vi "ControllerUI_New_with_command_read.vi"() -> ()   [LabVIEW 2026]
uses:
  <vilib>/Utility/error.llb/Trim Whitespace One-Sided.vi
panel:
  out "Numeric":i32
  out "after substring":string
  out "String":string
  out "script Status 3":string caption="script Status"
  out "script Status 2":string caption="script Status"
  in  "Percentage":dbl(slide) step=1.0 scale=0.0..100.0 scale format="%#.6g"
  out "IP":string="192.168.149.128"
  out "Port":dbl
  in  "BTN_DESD_3":bool
  in  "BTN_Grid_1":bool
  in  "BTN_Load_4":bool
  in  "BTN_Load_2":bool
  in  "BTN_Load_3":bool
  in  "BTN_Load_1":bool
  in  "BTN_DESD_2":bool
  in  "BTN_Gen_1":bool
  in  "BTN_PV_1":bool
  in  "BTN_Gen_2":bool
  in  "BTN_PV_2":bool
  in  "BTN_DESD_4":bool
  in  "BTN_DESD_1":bool
  in  "BTN_Wind_Turbine":bool
  out "background":picture
  in  "Tab Control":T1(tab)
  in  "Mode 4":bool
  in  "Mode 3":bool
  in  "Mode 2":bool
  in  "Mode 1：5-Day Rainstorm-to-Flood":bool
  out "script Status":string
  out "remaining text":string
  in  "String Control":string
  in  "PA1":dbl caption="Percentage (0-100)" min=0.0 max=30.0 step=0.5
  in  "stop":bool
  out "Local Status":string
  in  "PA3":dbl caption="Voltage 2 (0-255)" min=0.0 max=255.0 step=1.0
  out "Last Update":string
  out "UDP Frame":string
  out "Active Power":string
  out "Current":string
  out "Voltage":string
  in  "Reset Node":bool
  in  "Read Device State":bool
  in  "Send UDP Command":bool
  in  "PA2":dbl caption="Voltage 1 (0-255)" min=0.0 max=80.0 step=1.0
  in  "Voltage Command":dbl min=0.0 max=255.0 step=1.0
  in  "Node Enable":bool
  out "Device Badge":string
  out "Selected Summary":string
  out "Device Description":string
  out "Node ID":string
  out "Device Name":string
  # "Preset Disaster Mode"
  # "Selected Node Telemetry"
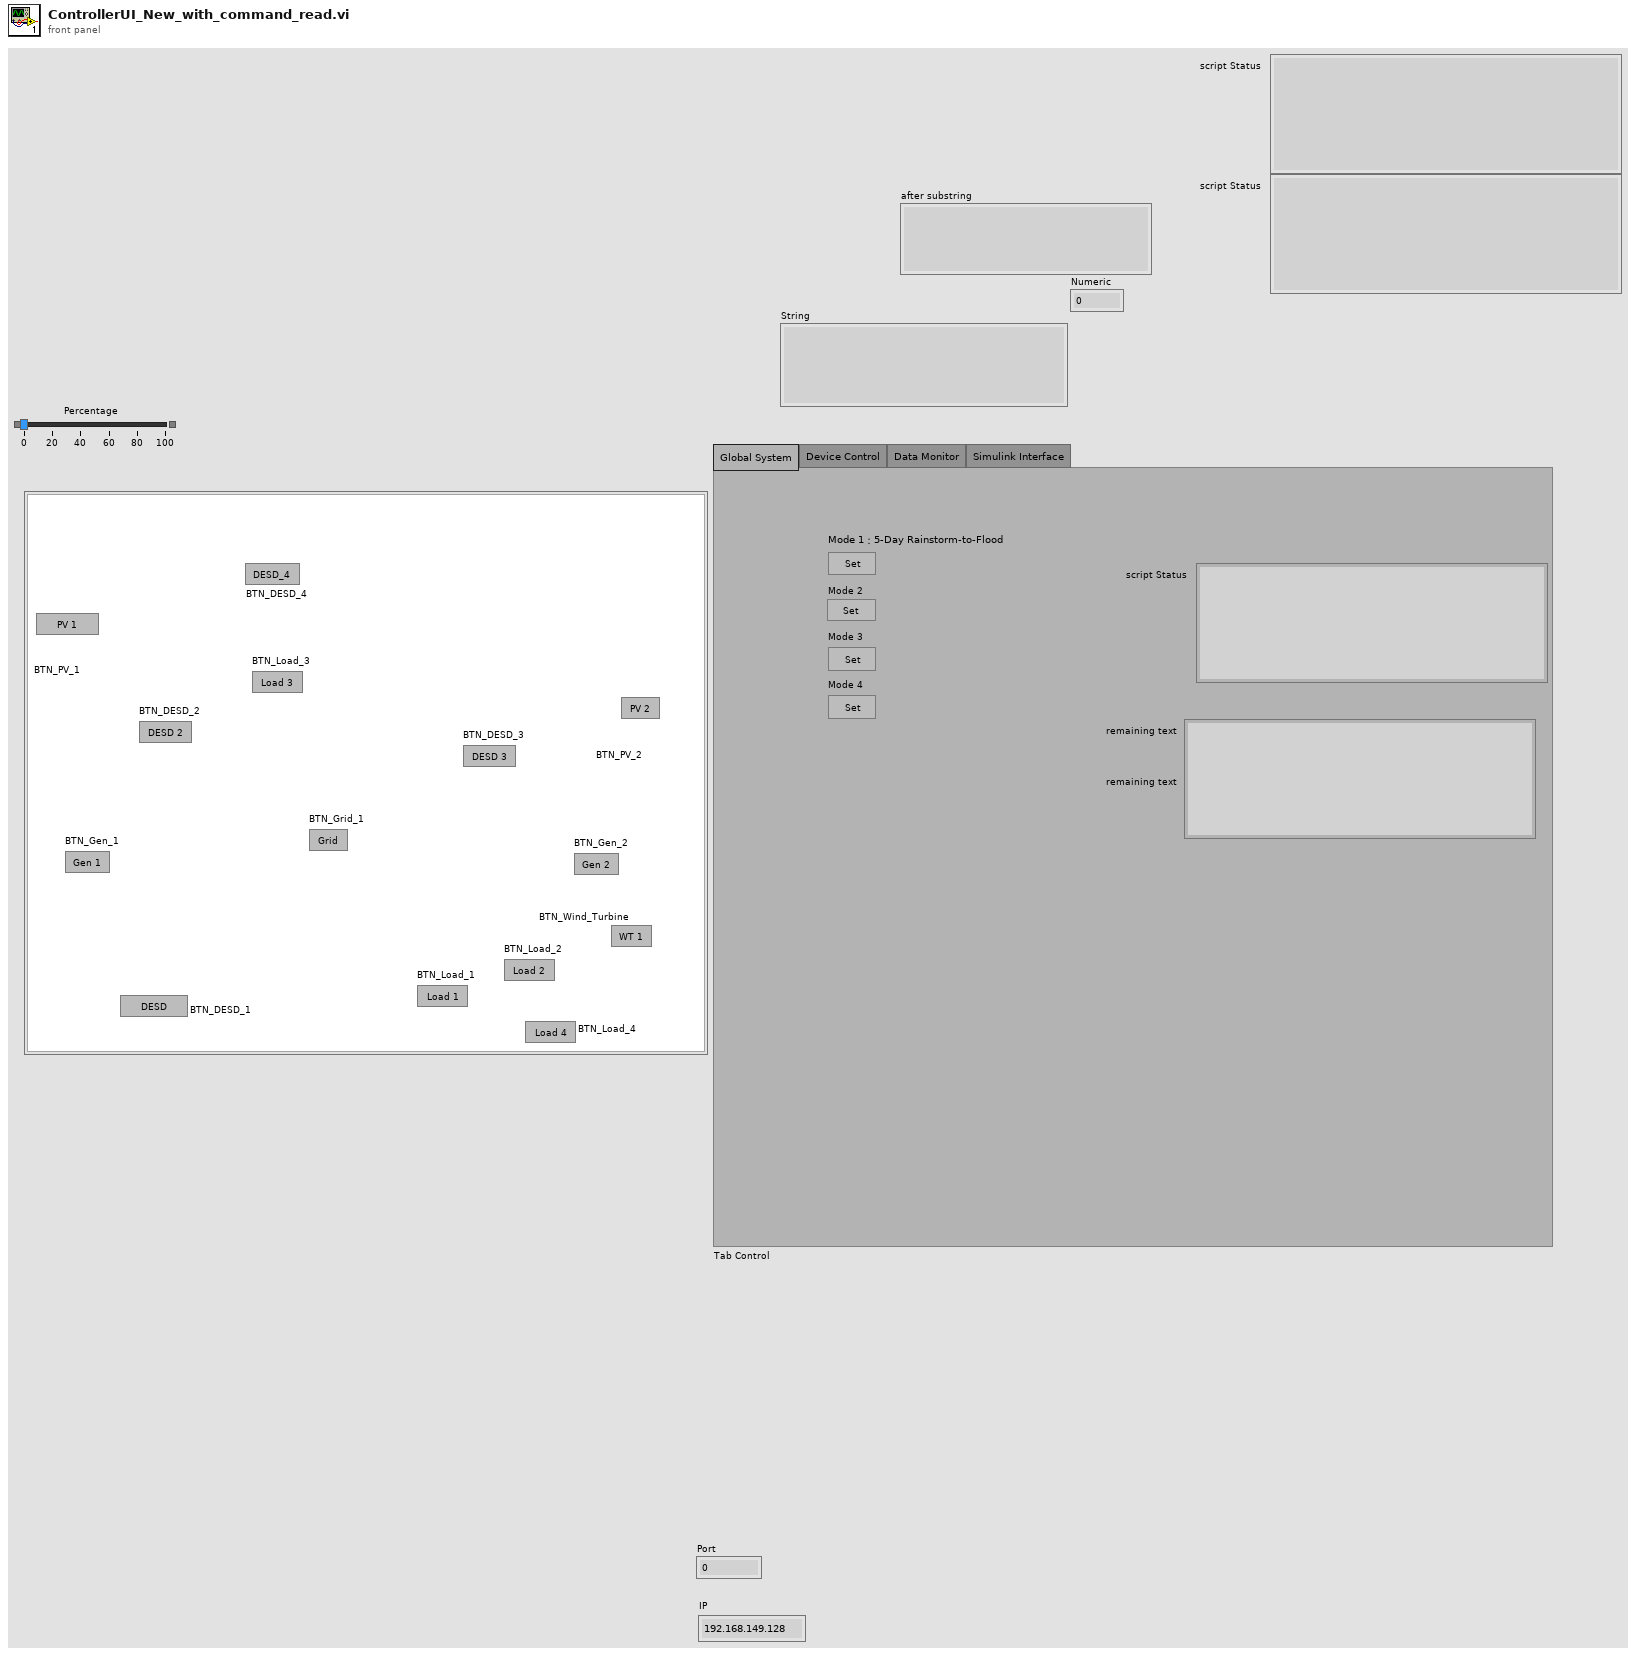
[diagram p1: front panel]
types:
  T1 = enum32{"Global System", "Device Control", "Data Monitor", "Simulink Interface"}
  T2 = typedef "imagedata.ctl" = cluster{"image type":i32, "image depth":i32, "image":u8[], "mask":u8[], "colors":u32[], "Rectangle":cluster{"left":i16, "top":i16, "right":i16, "bottom":i16}}
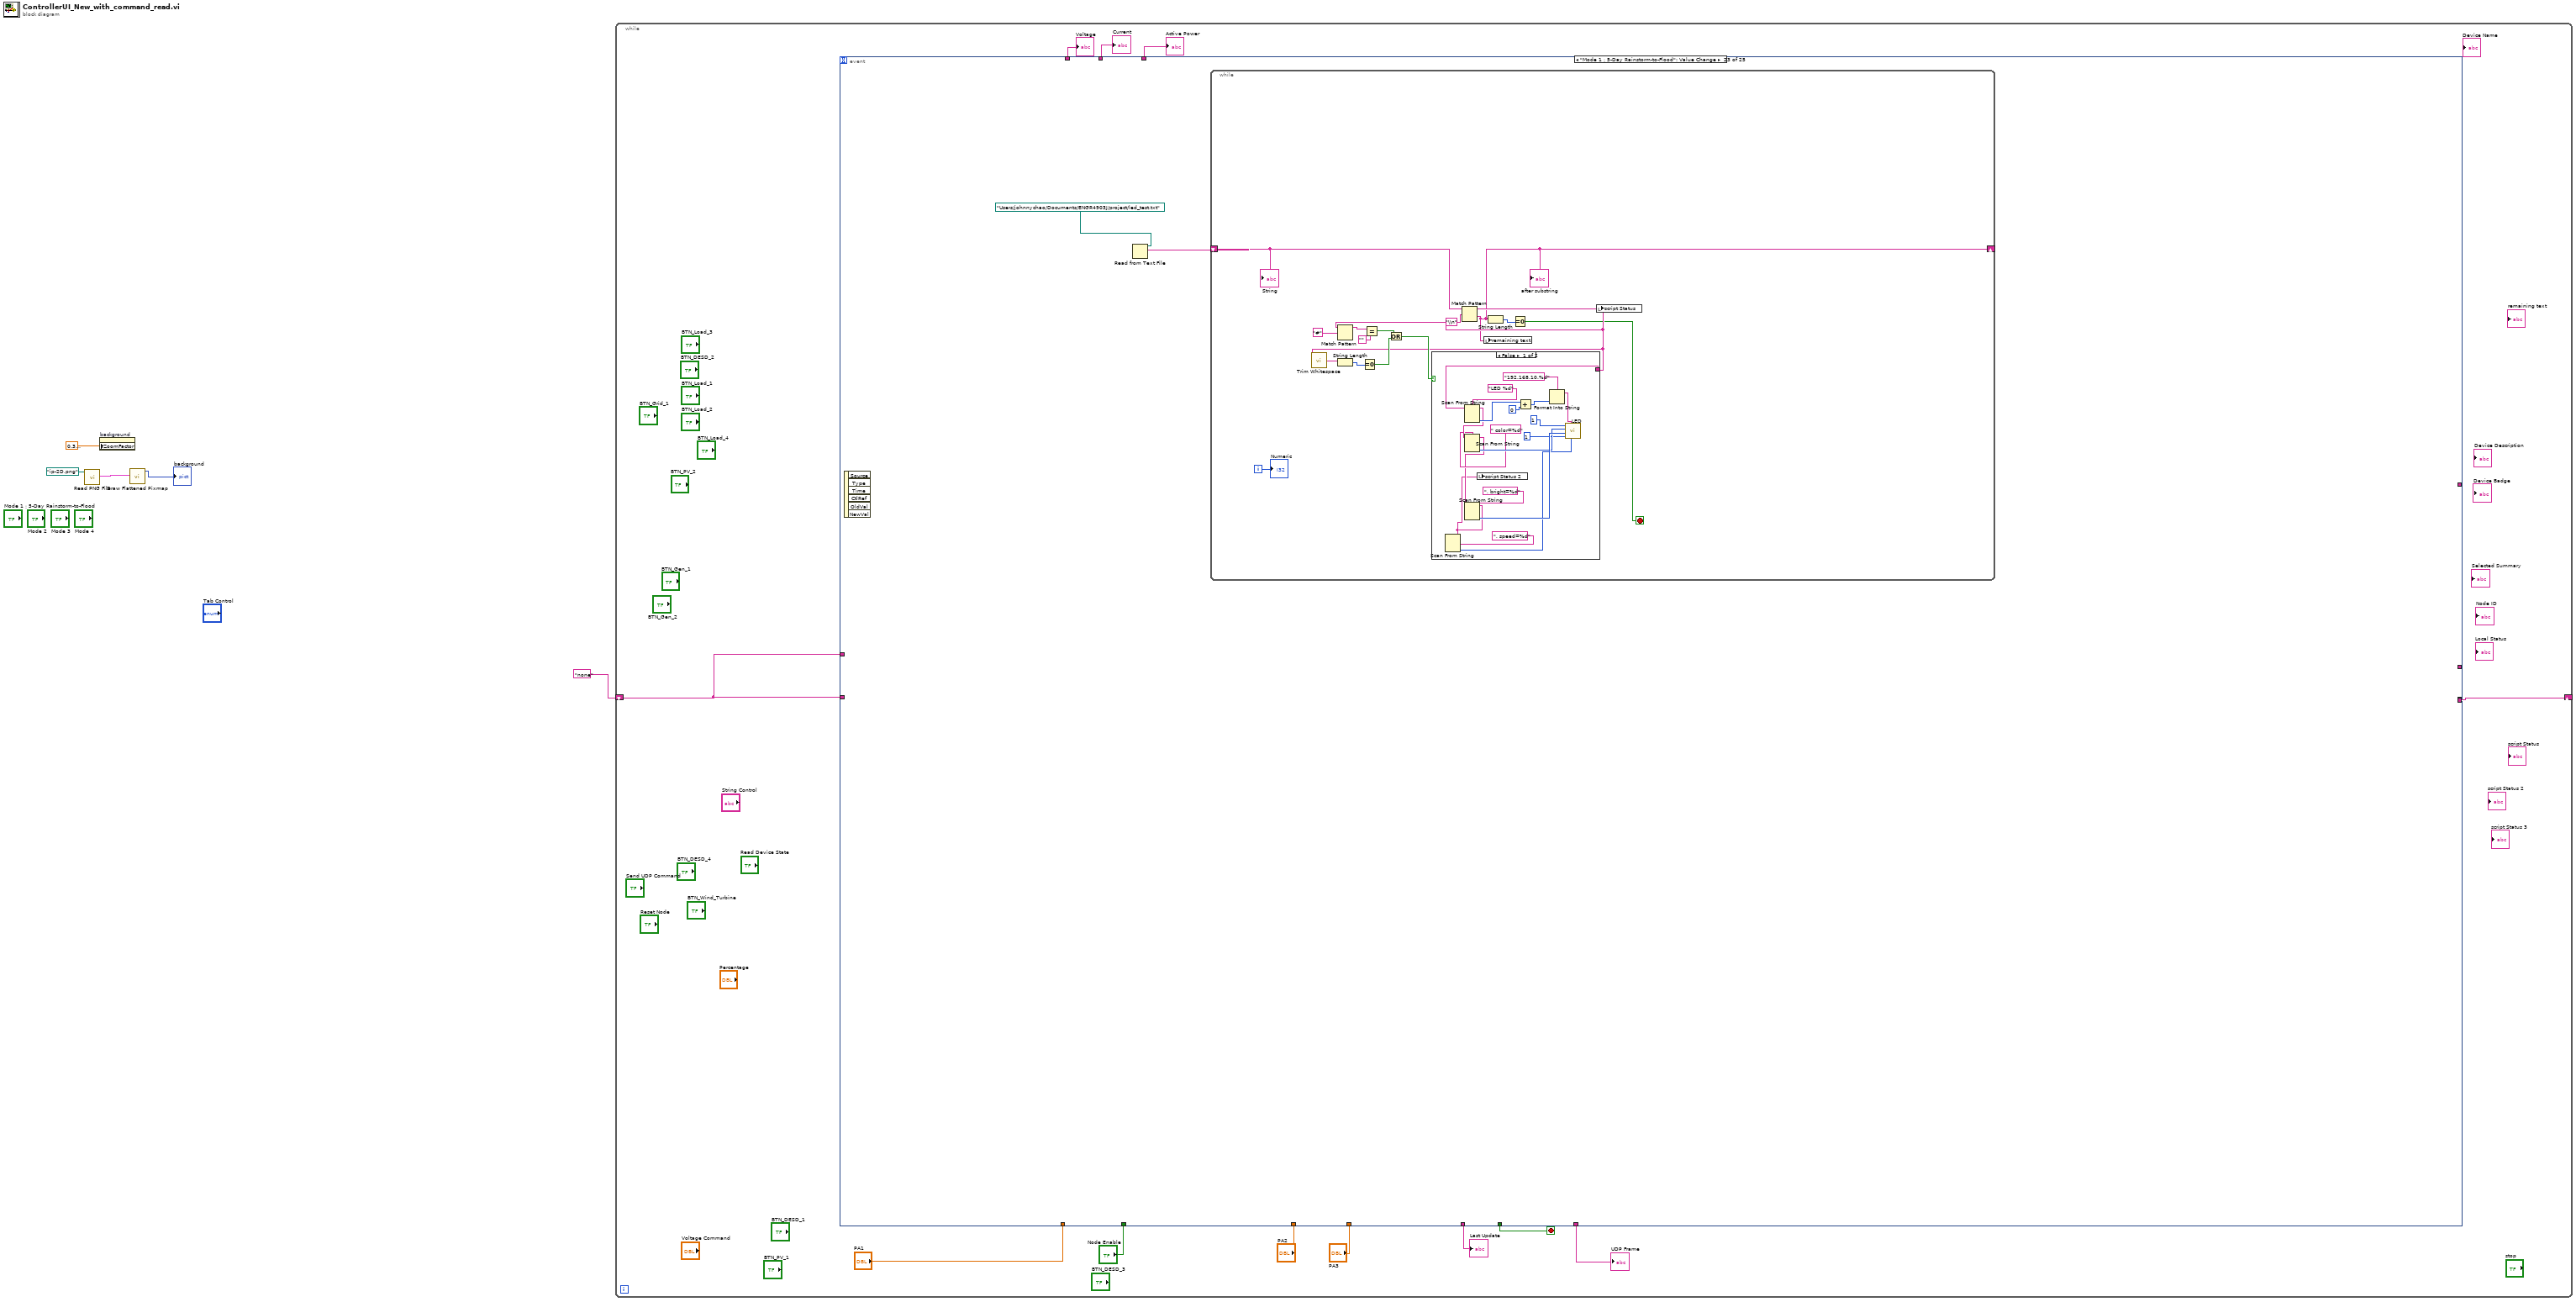
[diagram p0: block diagram]
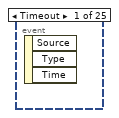
[diagram p2: hidden frame]
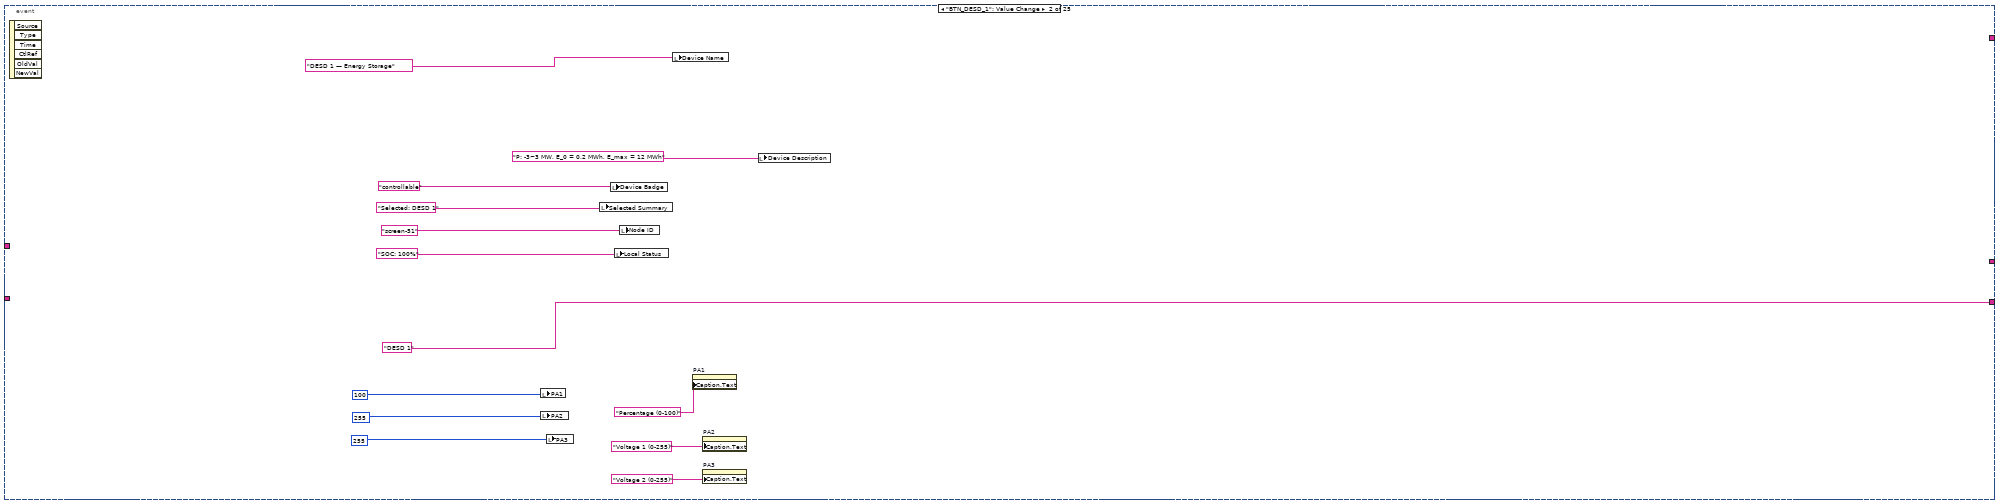
[diagram p3: hidden frame]
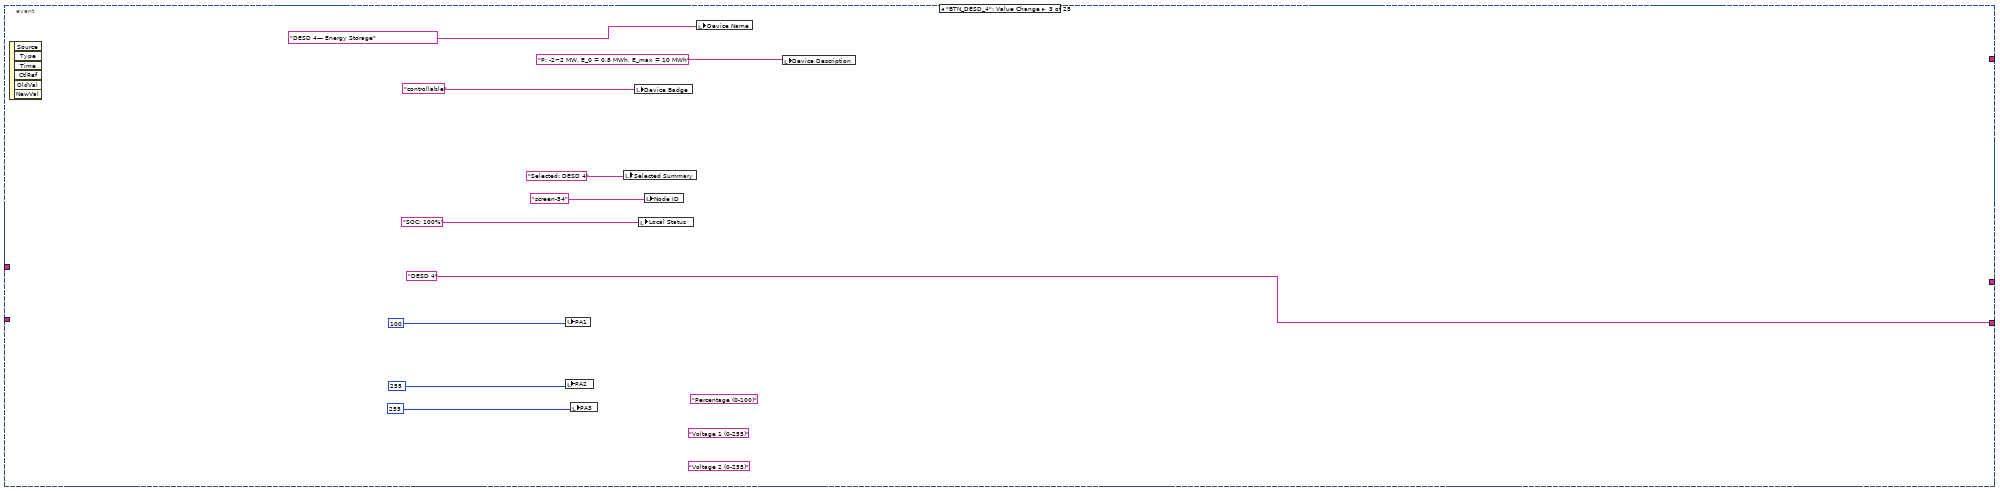
[diagram p4: hidden frame]
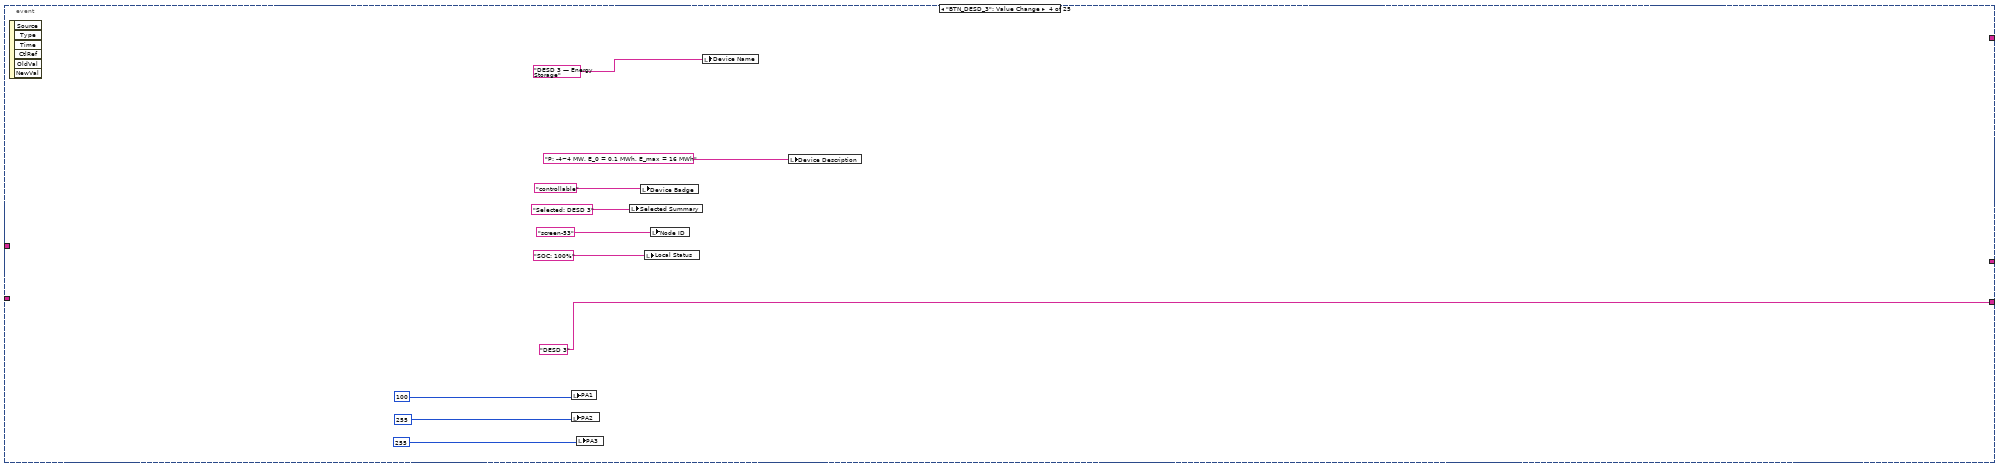
[diagram p5: hidden frame]
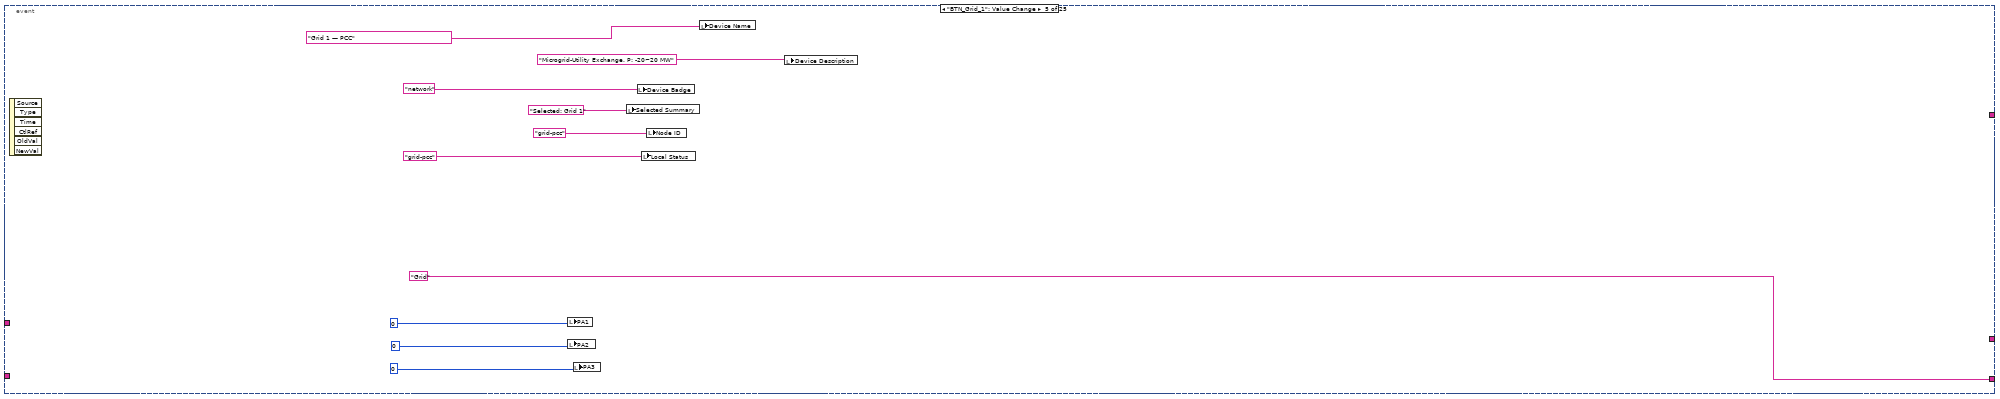
[diagram p6: hidden frame]
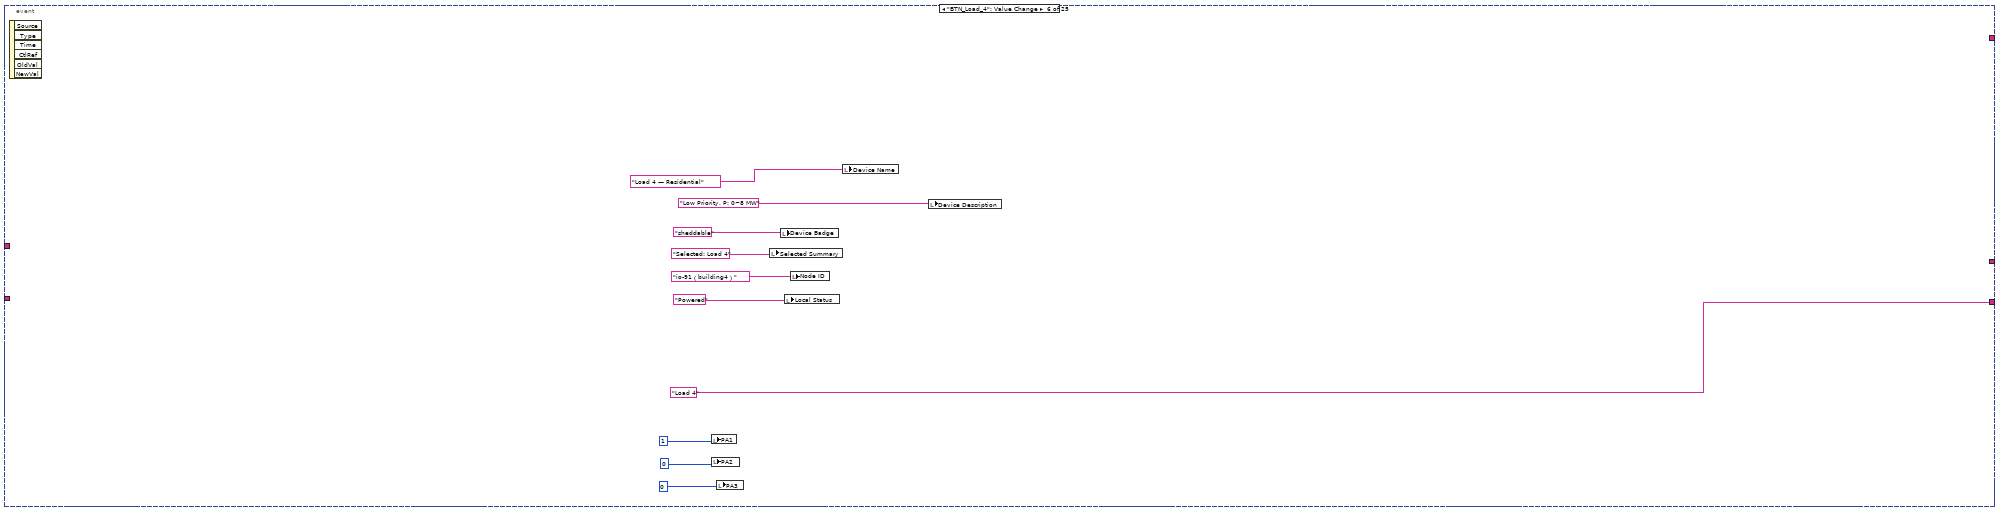
[diagram p7: hidden frame]
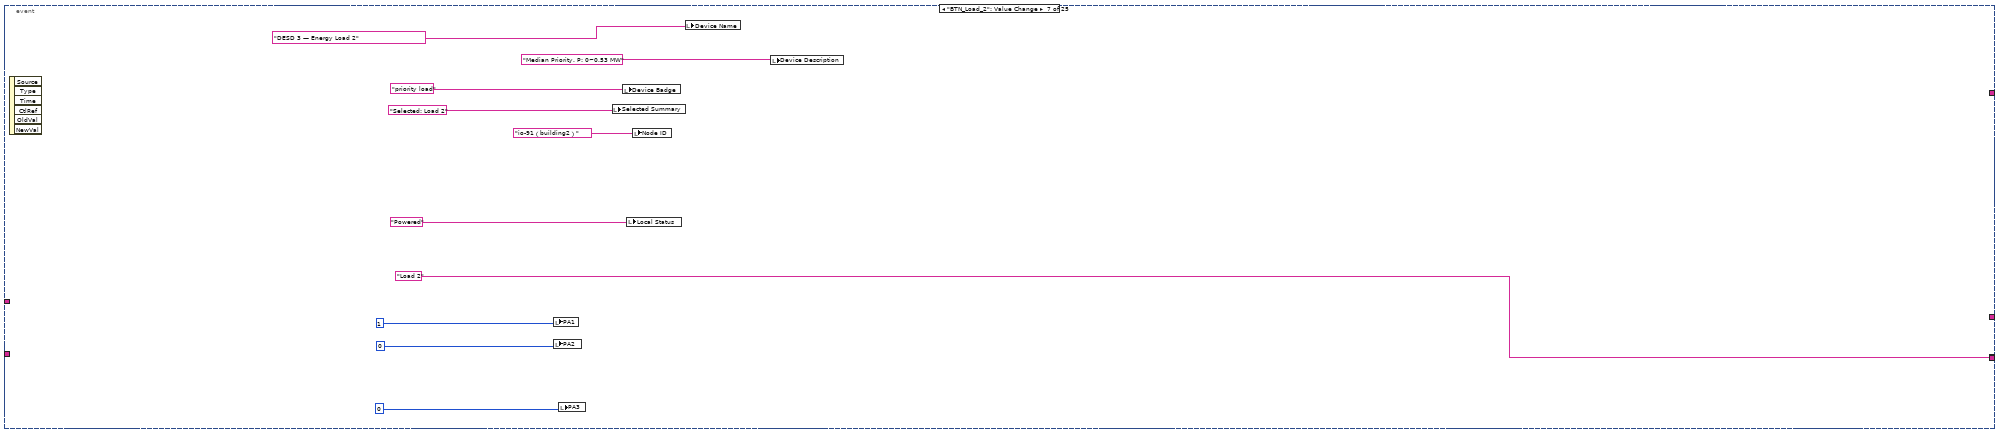
[diagram p8: hidden frame]
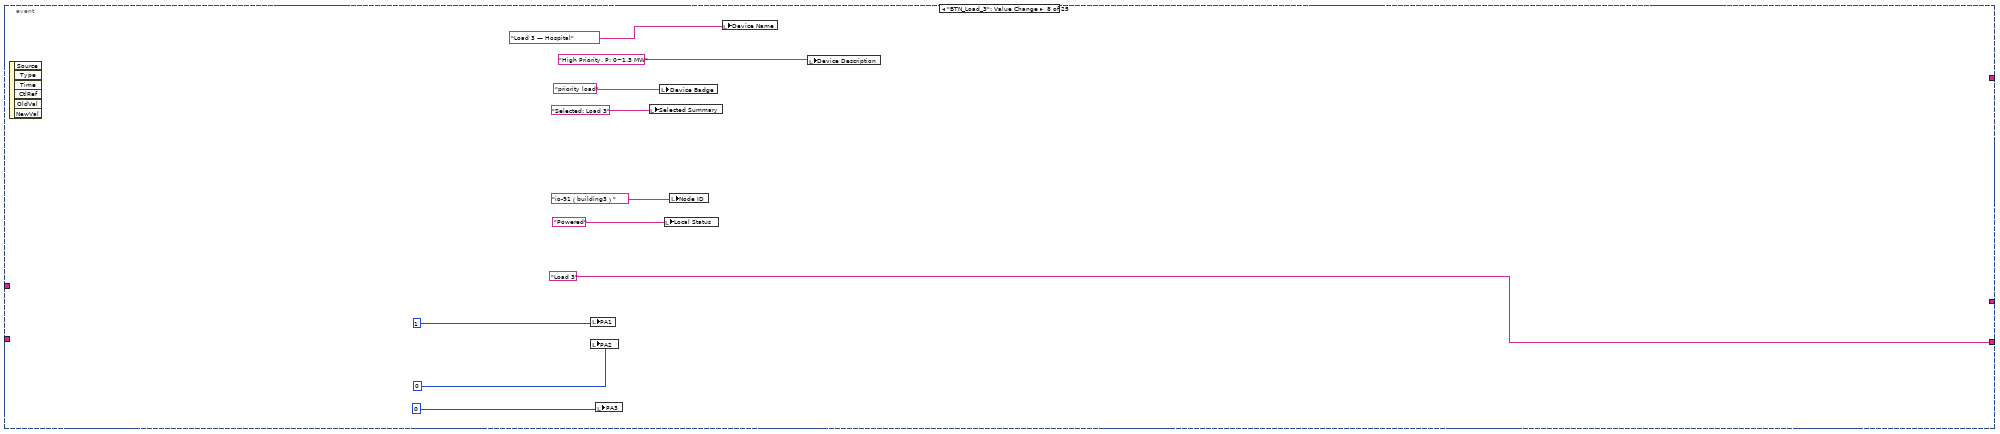
[diagram p9: hidden frame]
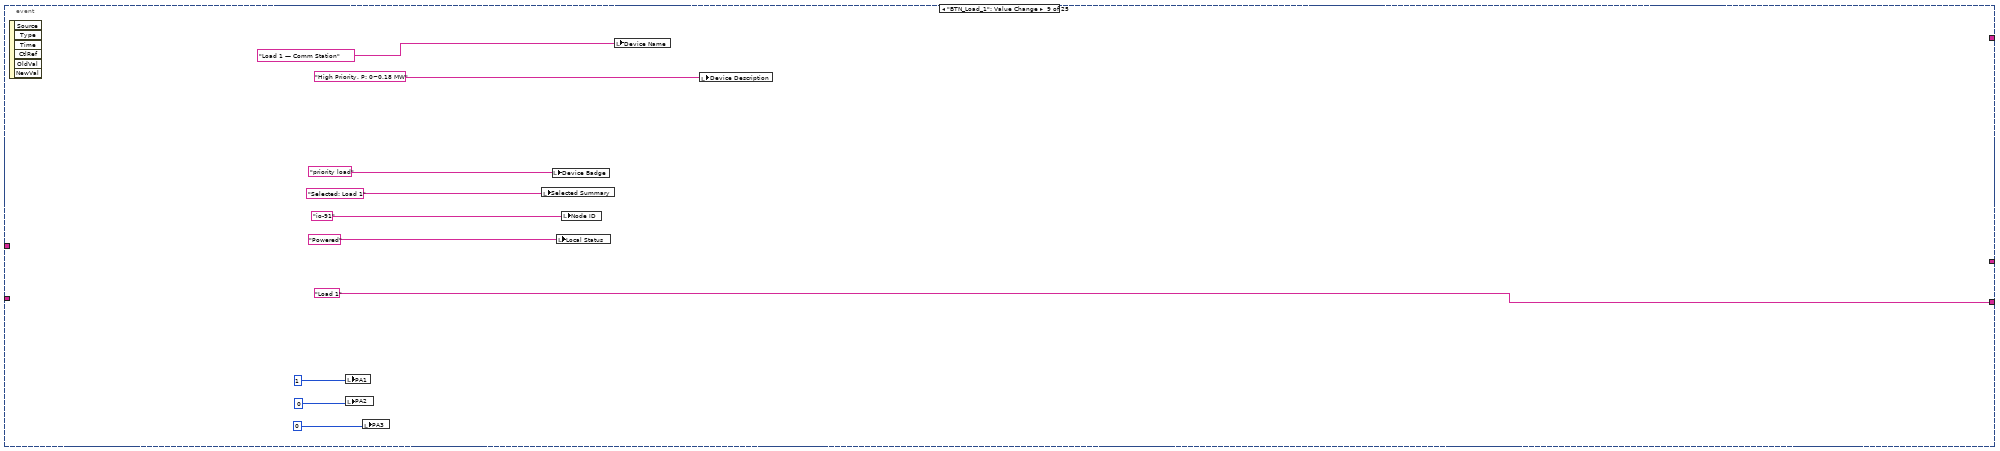
[diagram p10: hidden frame]
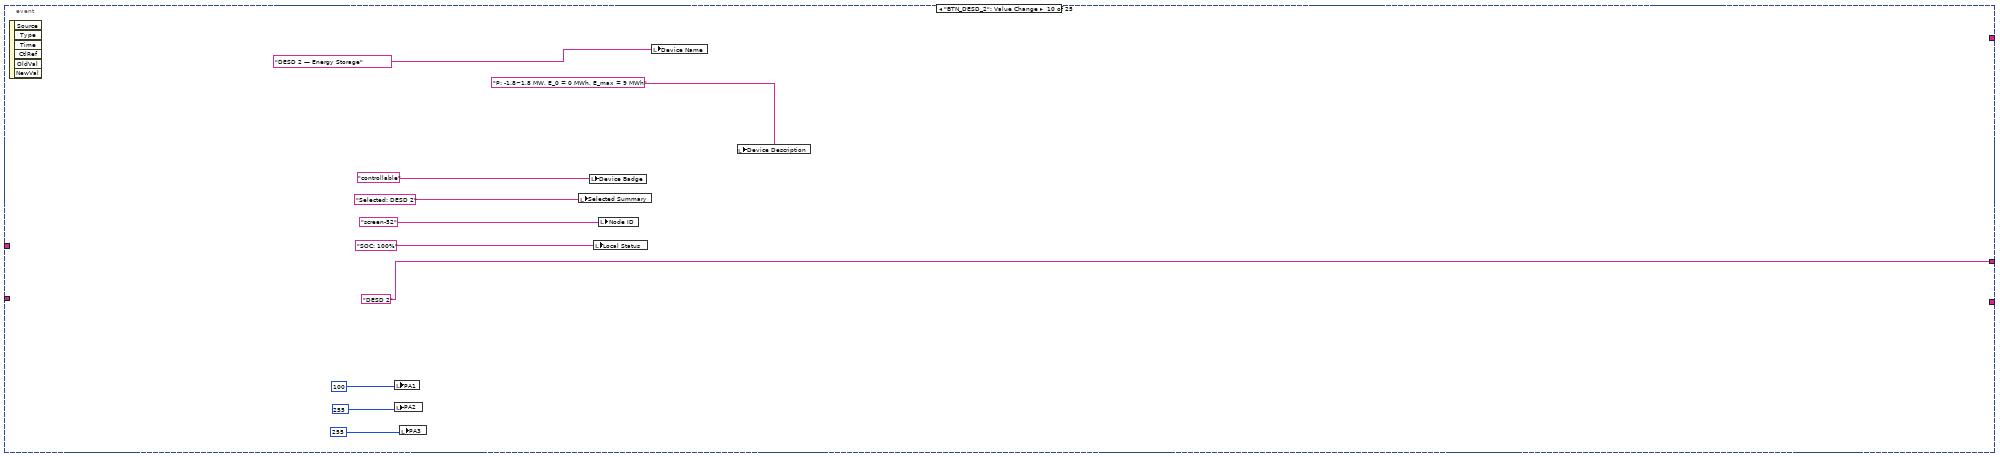
[diagram p11: hidden frame]
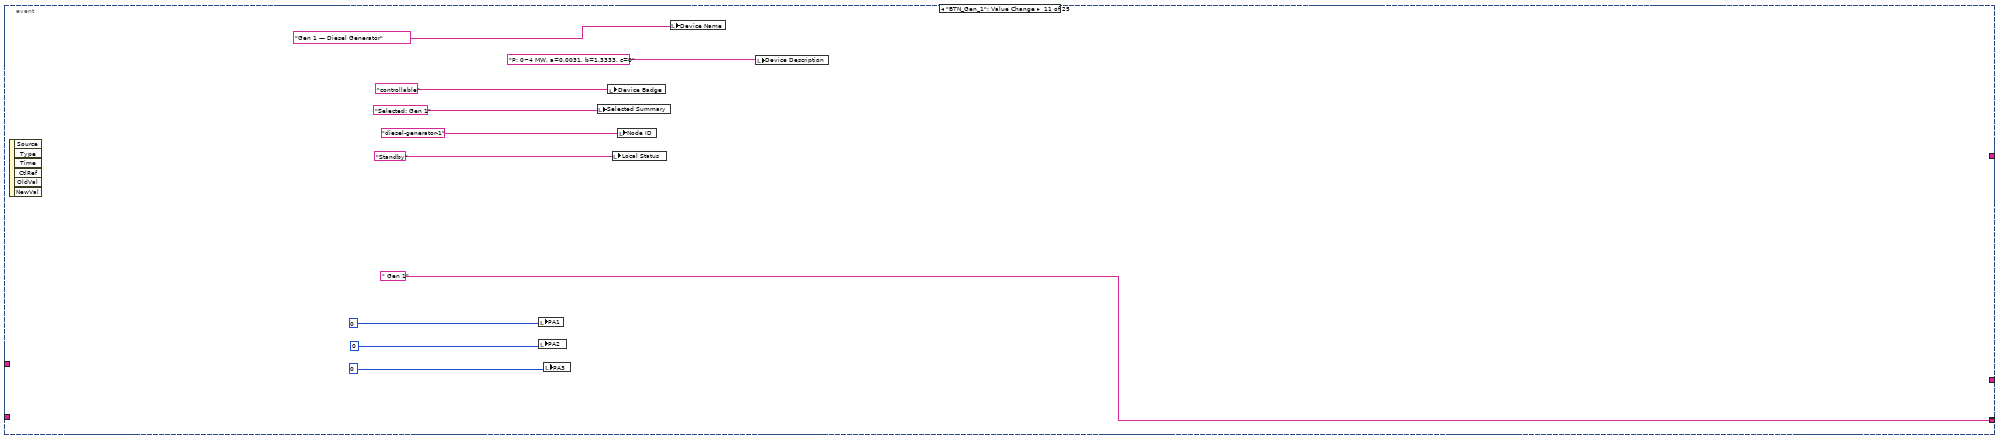
[diagram p12: hidden frame]
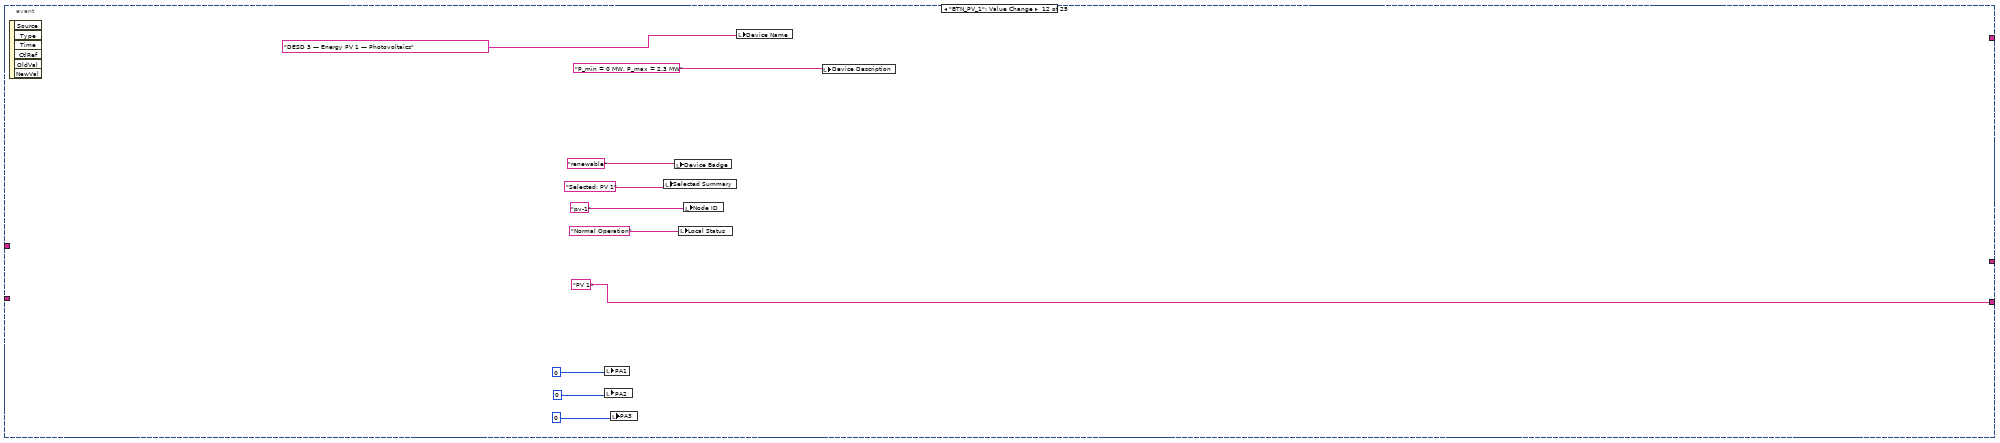
[diagram p13: hidden frame]
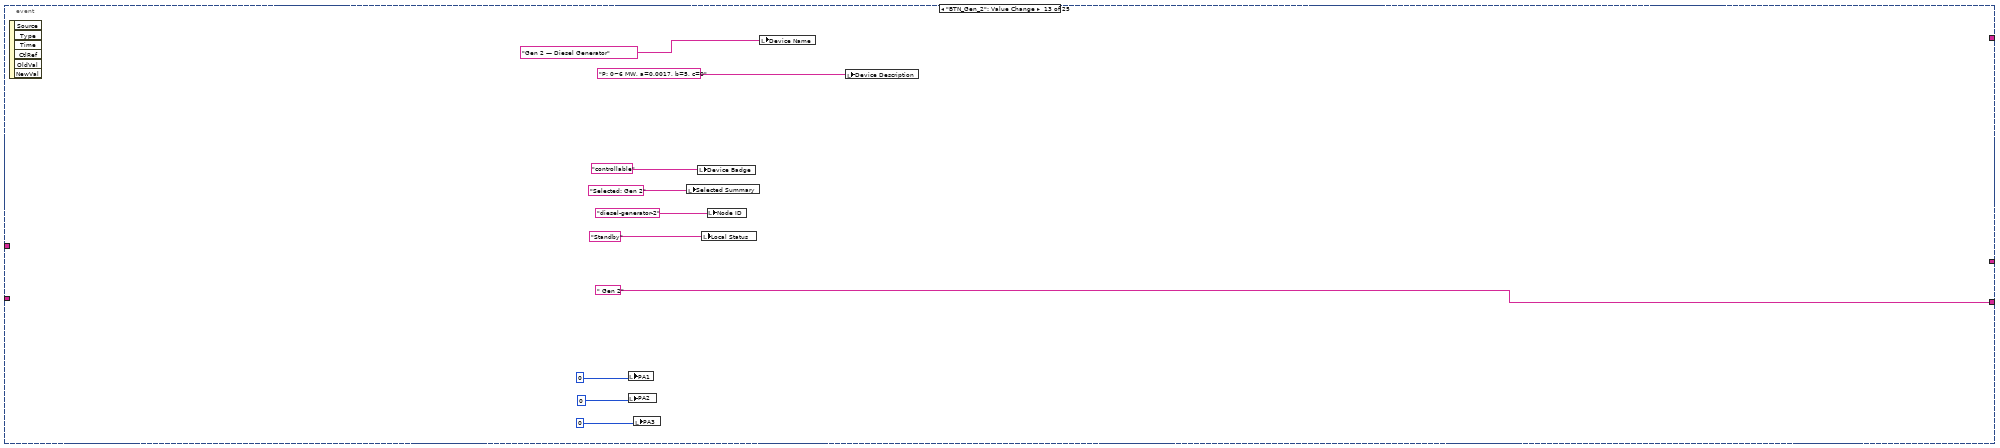
[diagram p14: hidden frame]
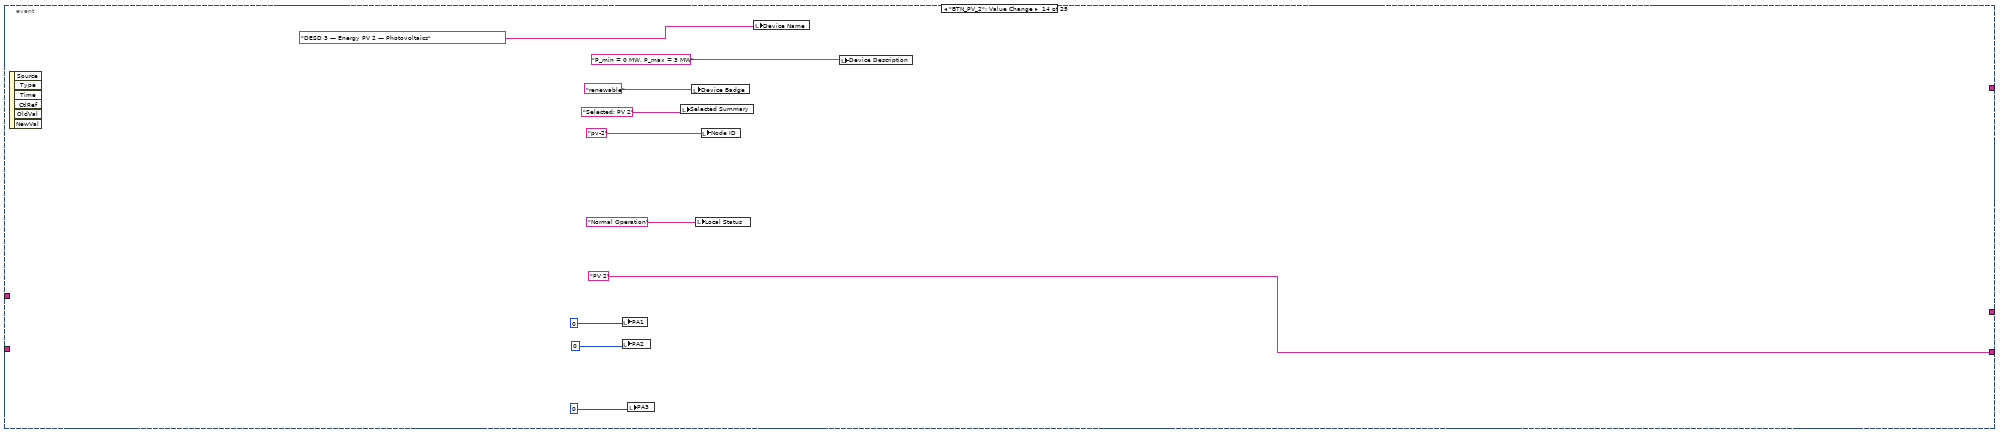
[diagram p15: hidden frame]
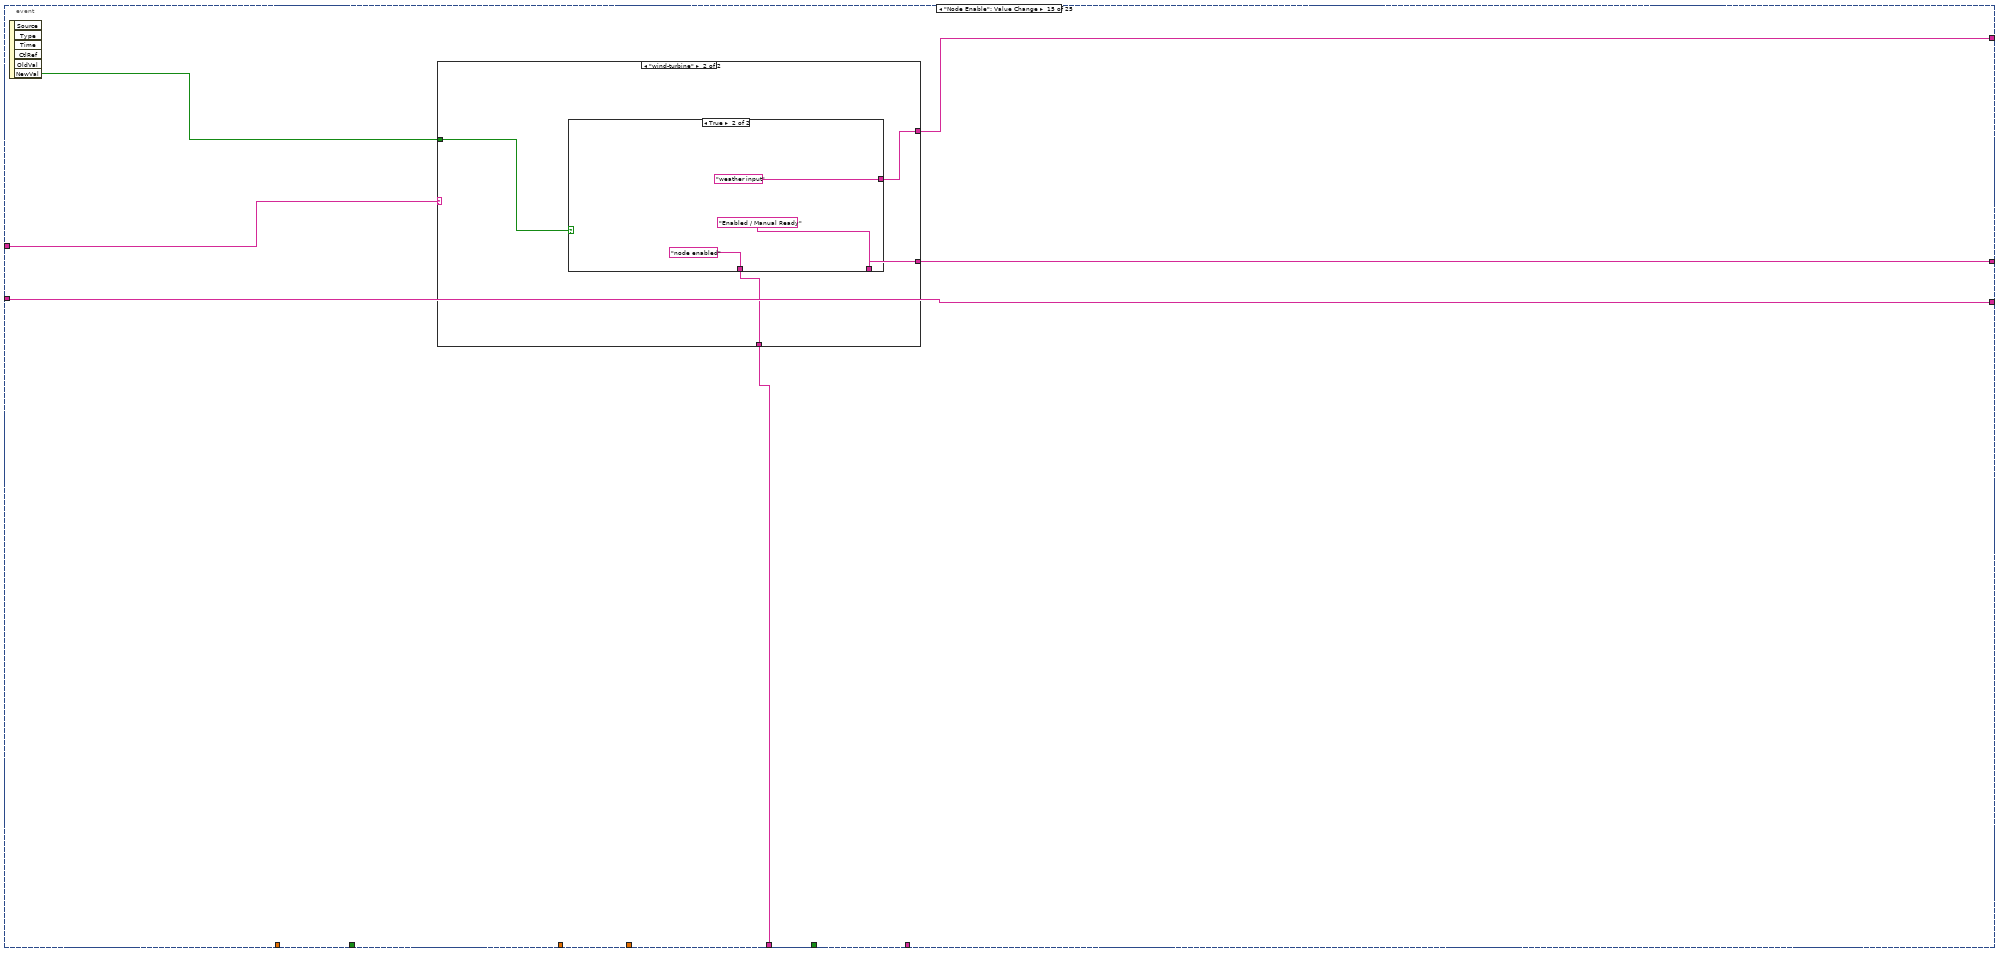
[diagram p16: hidden frame]
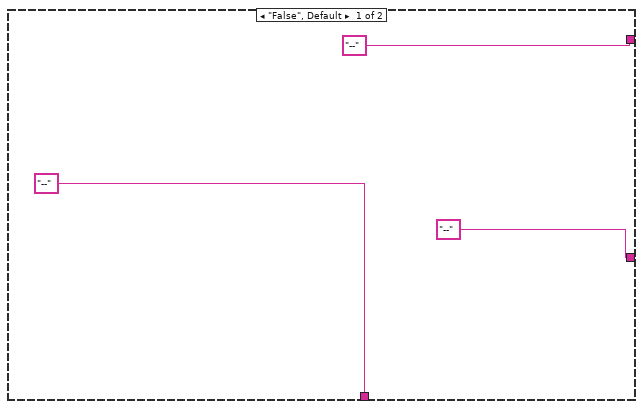
[diagram p17: hidden frame]
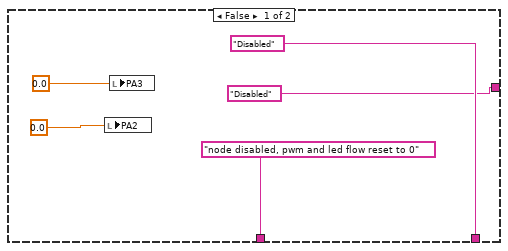
[diagram p18: hidden frame]
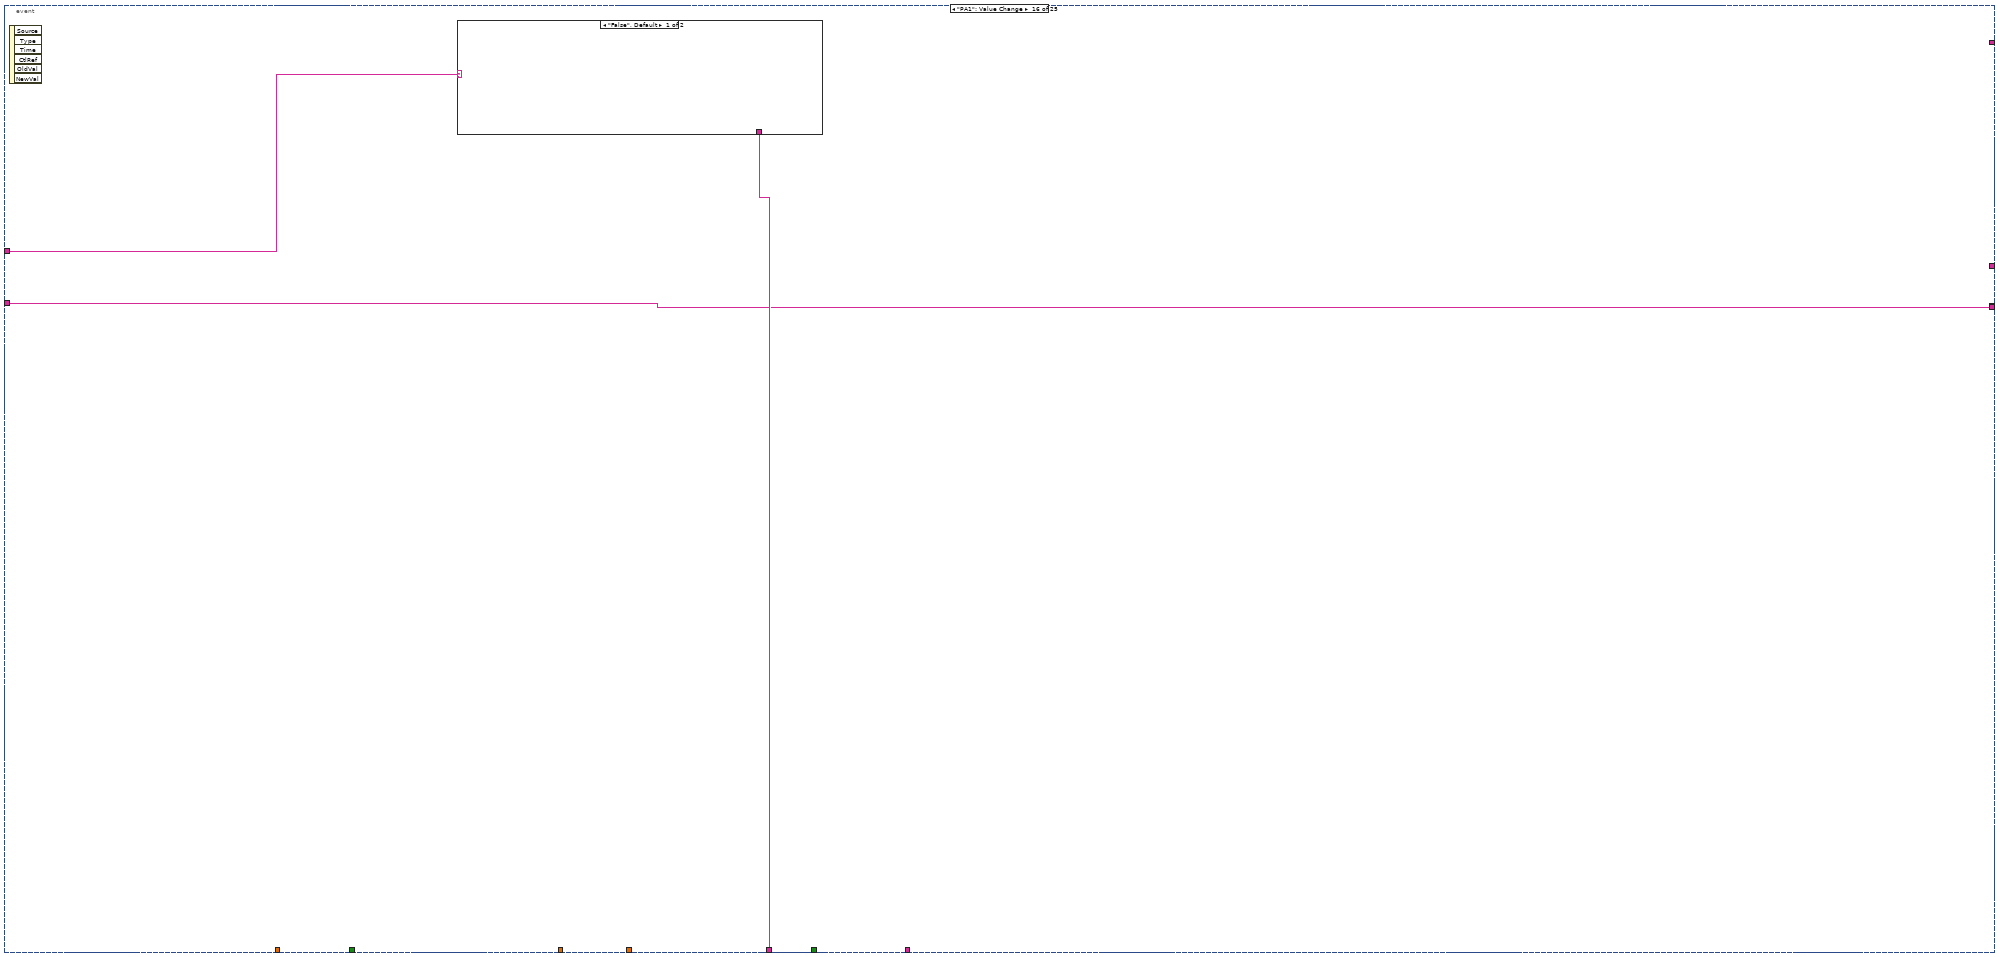
[diagram p19: hidden frame]
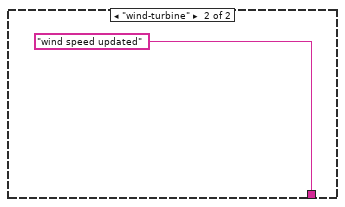
[diagram p20: hidden frame]
diagram:
  n1 = call <vilib>:"Read PNG File.vi"("path to PNG file"=path "ip-2D.png") -> ("image data"=w5:T2)  [unwired: 8 in, 2 out]
  n2 = property on="background" class="Pict"("ZoomFactor"=sgl 0.3 ("Zoom Factor")) -> ()  [unwired: 2 in, 2 out]
  n3 = call <vilib>:"Draw Flattened Pixmap.vi"("image data"=w5) -> ("new picture"=→"background":picture)  [unwired: 8 in]
  n4 = while {
    shift-right: [w7] -> _
    shift-left: "none" -> [w6]
    stop <- w17 stop-if-true
    n5 = event shown="[22] \"Mode 1：5-Day Rainstorm-to-Flood\": Value Change" {
      selector: _ -> [_ _ _ _ _ _ _ _ _ _ _ _ _ _ _ _ _ _ _ _ _ _ _ _ _]
      dyn-events: _ -> [_ _ _ _ _ _ _ _ _ _ _ _ _ _ _ _ _ _ _ _ _ _ _ _ _]
      timeout: _ -> [_ _ _ _ _ _ _ _ _ _ _ _ _ _ _ _ _ _ _ _ _ _ _ _ _]
      tunnel: [_ _ _ _ _ _ _ _ _ _ _ _ _ _ _ _ _ _ _ _ _ _ _ _ TRUE] -> w17
      tunnel: [_ _ _ _ _ _ _ _ _ "DESD 2" _ _ _ _ w154 _ _ _ w187 _ _ _ _ _ _] -> _
      tunnel: [_ _ _ _ _ _ _ _ _ _ _ _ _ _ w153 _ _ _ w186 _ _ _ _ _ _] -> _
      tunnel: [_ _ _ _ _ _ _ _ _ _ _ _ _ _ w155 w174 w178 w182 w188 w197 _ w266 _ _ _] -> w16
      tunnel: "Node Enable" -> [_ _ _ _ _ _ _ _ _ _ _ _ _ _ _ _ _ _ _ w202 _ _ _ _ _]
      tunnel: "PA1" -> [_ _ _ _ _ _ _ _ _ _ _ _ _ _ _ _ _ _ _ w201 _ _ _ _ _]
      tunnel: "PA3" -> [_ _ _ _ _ _ _ _ _ _ _ _ _ _ _ _ _ _ _ w200 _ _ _ _ _]
      tunnel: "PA2" -> [_ _ _ _ _ _ _ _ _ _ _ _ _ _ _ _ _ _ _ w199 _ _ _ _ _]
      tunnel: [_ _ _ _ _ _ _ _ _ _ _ _ _ _ _ _ _ _ _ w198 _ _ _ _ _] -> w11
      tunnel: [_ _ _ _ _ _ _ _ _ _ _ _ _ _ _ _ _ _ _ _ _ w265 _ _ _] -> w10
      tunnel: [_ _ _ _ _ _ _ _ _ _ _ _ _ _ _ _ _ _ _ _ _ w264 _ _ _] -> w9
      tunnel: [_ _ _ _ _ _ _ _ _ _ _ _ _ _ _ _ _ _ _ _ _ w263 _ _ _] -> w8
      tunnel: [_ "DESD 1" "DESD 4" "DESD 3" "Grid" "Load 4" "Load 2" "Load 3" "Load 1" _ " Gen 1" "PV 1" " Gen 2" _ w151 _ w176 w180 _ w196 "wind-turbine" w261 _ _ w337] -> w7
      tunnel: w6 -> [_ _ _ _ _ _ _ _ _ _ _ _ _ _ w152 w173 w177 w181 w185 w196 _ w262 _ _ _]
      tunnel: w6 -> [_ _ _ _ _ _ _ _ _ _ _ _ _ _ w151 w172 w176 w180 w184 _ _ w261 _ _ w337]
      tunnel: [_ _ _ _ _ _ _ _ _ _ _ _ _ "PV 2" _ w172 _ _ _ _ _ _ _ _ _] -> _
      tunnel: [_ _ _ _ _ _ _ _ _ _ _ _ _ _ _ _ _ _ w184 _ _ _ _ _ _] -> _
      event Timeout {
        n6 = event-data() -> ()  [unwired: 1 in, 3 out]
      }
      event "BTN_DESD_1": Value Change {
        n7 = event-data() -> ()  [unwired: 1 in, 6 out]
        n8 = local write "PA1"(100) -> ()
        n9 = local write "PA2"(255) -> ()
        n10 = local write "PA3"(255) -> ()
        n11 = local write "Selected Summary"("Selected: DESD 1") -> ()
        n12 = local write "Device Badge"("controllable") -> ()
        n13 = local write "Local Status"("SOC: 100%") -> ()
        n14 = local write "Node ID"("screen-51") -> ()
        n15 = local write "Device Name"("DESD 1 — Energy Storage") -> ()
        n16 = property on="PA1" class="DigNum (strict)"("Caption.Text"="Percentage (0-100)") -> ()  [unwired: 2 in, 2 out]
        n17 = property on="PA2" class="DigNum (strict)"("Caption.Text"="Voltage 1 (0-255)") -> ()  [unwired: 2 in, 2 out]
        n18 = property on="PA3" class="DigNum (strict)"("Caption.Text"="Voltage 2 (0-255)") -> ()  [unwired: 2 in, 2 out]
        n19 = local write "Device Description"("P: -3~3 MW, E_0 = 0.2 MWh, E_max = 12 MWh") -> ()
      }
      event "BTN_DESD_4": Value Change {
        (unwired) "Voltage 2 (0-255)"
        (unwired) "Voltage 1 (0-255)"
        (unwired) "Percentage (0-100)"
        n20 = event-data() -> ()  [unwired: 1 in, 6 out]
        n21 = local write "PA1"(100) -> ()
        n22 = local write "PA2"(255) -> ()
        n23 = local write "PA3"(255) -> ()
        n24 = local write "Selected Summary"("Selected: DESD 4") -> ()
        n25 = local write "Device Badge"("controllable") -> ()
        n26 = local write "Local Status"("SOC: 100%") -> ()
        n27 = local write "Node ID"("screen-54") -> ()
        n28 = local write "Device Name"("DESD 4— Energy Storage") -> ()
        n29 = local write "Device Description"("P: -2~2 MW, E_0 = 0.8 MWh, E_max = 10 MWh") -> ()
      }
      event "BTN_DESD_3": Value Change {
        n30 = event-data() -> ()  [unwired: 1 in, 6 out]
        n31 = local write "PA1"(100) -> ()
        n32 = local write "PA2"(255) -> ()
        n33 = local write "PA3"(255) -> ()
        n34 = local write "Selected Summary"("Selected: DESD 3") -> ()
        n35 = local write "Device Badge"("controllable") -> ()
        n36 = local write "Local Status"("SOC: 100%") -> ()
        n37 = local write "Node ID"("screen-53") -> ()
        n38 = local write "Device Name"("DESD 3 — Energy Storage") -> ()
        n39 = local write "Device Description"("P: -4~4 MW, E_0 = 0.1 MWh, E_max = 16 MWh") -> ()
      }
      event "BTN_Grid_1": Value Change {
        n40 = event-data() -> ()  [unwired: 1 in, 6 out]
        n41 = local write "PA1"(0) -> ()
        n42 = local write "PA2"(0) -> ()
        n43 = local write "PA3"(0) -> ()
        n44 = local write "Selected Summary"("Selected: Grid 1") -> ()
        n45 = local write "Device Badge"("network") -> ()
        n46 = local write "Local Status"("grid-pcc") -> ()
        n47 = local write "Node ID"("grid-pcc") -> ()
        n48 = local write "Device Name"("Grid 1 — PCC") -> ()
        n49 = local write "Device Description"("Microgrid-Utility Exchange. P: -20~20 MW") -> ()
      }
      event "BTN_Load_4": Value Change {
        n50 = event-data() -> ()  [unwired: 1 in, 6 out]
        n51 = local write "PA1"(1) -> ()
        n52 = local write "PA2"(0) -> ()
        n53 = local write "PA3"(0) -> ()
        n54 = local write "Selected Summary"("Selected: Load 4") -> ()
        n55 = local write "Device Badge"("sheddable") -> ()
        n56 = local write "Local Status"("Powered") -> ()
        n57 = local write "Node ID"("io-91（building4）") -> ()
        n58 = local write "Device Name"("Load 4 — Residential") -> ()
        n59 = local write "Device Description"("Low Priority. P: 0~8 MW") -> ()
      }
      event "BTN_Load_2": Value Change {
        n60 = event-data() -> ()  [unwired: 1 in, 6 out]
        n61 = local write "PA1"(1) -> ()
        n62 = local write "PA2"(0) -> ()
        n63 = local write "PA3"(0) -> ()
        n64 = local write "Selected Summary"("Selected: Load 2") -> ()
        n65 = local write "Device Badge"("priority load") -> ()
        n66 = local write "Local Status"("Powered") -> ()
        n67 = local write "Node ID"("io-91（building2）") -> ()
        n68 = local write "Device Name"("DESD 3 — Energy Load 2") -> ()
        n69 = local write "Device Description"("Median Priority. P: 0~0.53 MW") -> ()
      }
      event "BTN_Load_3": Value Change {
        n70 = event-data() -> ()  [unwired: 1 in, 6 out]
        n71 = local write "PA1"(1) -> ()
        n72 = local write "PA2"(0) -> ()
        n73 = local write "PA3"(0) -> ()
        n74 = local write "Selected Summary"("Selected: Load 3") -> ()
        n75 = local write "Device Badge"("priority load") -> ()
        n76 = local write "Local Status"("Powered") -> ()
        n77 = local write "Node ID"("io-91（building3）") -> ()
        n78 = local write "Device Name"("Load 3 — Hospital") -> ()
        n79 = local write "Device Description"("High Priority. P: 0~1.3 MW") -> ()
      }
      event "BTN_Load_1": Value Change {
        n80 = event-data() -> ()  [unwired: 1 in, 6 out]
        n81 = local write "PA1"(1) -> ()
        n82 = local write "PA2"(0) -> ()
        n83 = local write "PA3"(0) -> ()
        n84 = local write "Selected Summary"("Selected: Load 1") -> ()
        n85 = local write "Device Badge"("priority load") -> ()
        n86 = local write "Local Status"("Powered") -> ()
        n87 = local write "Node ID"("io-91") -> ()
        n88 = local write "Device Name"("Load 1 — Comm Station") -> ()
        n89 = local write "Device Description"("High Priority. P: 0~0.18 MW") -> ()
      }
      event "BTN_DESD_2": Value Change {
        n90 = event-data() -> ()  [unwired: 1 in, 6 out]
        n91 = local write "PA1"(100) -> ()
        n92 = local write "PA2"(255) -> ()
        n93 = local write "PA3"(255) -> ()
        n94 = local write "Selected Summary"("Selected: DESD 2") -> ()
        n95 = local write "Device Badge"("controllable") -> ()
        n96 = local write "Local Status"("SOC: 100%") -> ()
        n97 = local write "Node ID"("screen-52") -> ()
        n98 = local write "Device Name"("DESD 2 — Energy Storage") -> ()
        n99 = local write "Device Description"("P: -1.8~1.8 MW, E_0 = 0 MWh, E_max = 9 MWh") -> ()
      }
      event "BTN_Gen_1": Value Change {
        n100 = event-data() -> ()  [unwired: 1 in, 6 out]
        n101 = local write "PA1"(0) -> ()
        n102 = local write "PA2"(0) -> ()
        n103 = local write "PA3"(0) -> ()
        n104 = local write "Selected Summary"("Selected: Gen 1") -> ()
        n105 = local write "Device Badge"("controllable") -> ()
        n106 = local write "Local Status"("Standby") -> ()
        n107 = local write "Node ID"("diesel-generator-1") -> ()
        n108 = local write "Device Name"("Gen 1 — Diesel Generator") -> ()
        n109 = local write "Device Description"("P: 0~4 MW, a=0.0031, b=1.3333, c=0") -> ()
      }
      event "BTN_PV_1": Value Change {
        n110 = event-data() -> ()  [unwired: 1 in, 6 out]
        n111 = local write "PA1"(0) -> ()
        n112 = local write "PA2"(0) -> ()
        n113 = local write "PA3"(0) -> ()
        n114 = local write "Selected Summary"("Selected: PV 1") -> ()
        n115 = local write "Device Badge"("renewable") -> ()
        n116 = local write "Local Status"("Normal Operation") -> ()
        n117 = local write "Node ID"("pv-1") -> ()
        n118 = local write "Device Name"("DESD 3 — Energy PV 1 — Photovoltaics") -> ()
        n119 = local write "Device Description"("P_min = 0 MW, P_max = 2.3 MW") -> ()
      }
      event "BTN_Gen_2": Value Change {
        n120 = event-data() -> ()  [unwired: 1 in, 6 out]
        n121 = local write "PA1"(0) -> ()
        n122 = local write "PA2"(0) -> ()
        n123 = local write "PA3"(0) -> ()
        n124 = local write "Selected Summary"("Selected: Gen 2") -> ()
        n125 = local write "Device Badge"("controllable") -> ()
        n126 = local write "Local Status"("Standby") -> ()
        n127 = local write "Node ID"("diesel-generator-2") -> ()
        n128 = local write "Device Name"("Gen 2 — Diesel Generator") -> ()
        n129 = local write "Device Description"("P: 0~6 MW, a=0.0017, b=5, c=0") -> ()
      }
      event "BTN_PV_2": Value Change {
        n130 = event-data() -> ()  [unwired: 1 in, 6 out]
        n131 = local write "PA1"(0) -> ()
        n132 = local write "PA2"(0) -> ()
        n133 = local write "PA3"(0) -> ()
        n134 = local write "Selected Summary"("Selected: PV 2") -> ()
        n135 = local write "Device Badge"("renewable") -> ()
        n136 = local write "Local Status"("Normal Operation") -> ()
        n137 = local write "Node ID"("pv-2") -> ()
        n138 = local write "Device Name"("DESD 3 — Energy PV 2 — Photovoltaics") -> ()
        n139 = local write "Device Description"("P_min = 0 MW, P_max = 3 MW") -> ()
      }
      event "Node Enable": Value Change {
        n140 = event-data() -> ("NewVal"=w156:bool)  [unwired: 1 in, 5 out]
        n141 = case shown="\"wind-turbine\"" w152 {
          tunnel: w156 -> [_ w163]
          tunnel: ["--" w162] -> w155
          tunnel: ["--" w161] -> w154
          tunnel: ["--" w160] -> w153
          frame "False", Default {
          }
          frame "wind-turbine" {
            n142 = case shown="True" w163 {
              tunnel: ["node disabled, pwm and led flow reset to 0" "node enabled"] -> w162
              tunnel: ["Disabled" "Enabled / Manual Ready"] -> w161
              tunnel: ["Disabled" "weather input"] -> w160
              frame False {
                n143 = local write "PA2"(0.0 ("WT Wind Speed")) -> ()
                n144 = local write "PA3"(0.0 ("WT PWM Command")) -> ()
              }
              frame True {
              }
            }
          }
        }
      }
      event "PA1": Value Change {
        n145 = event-data() -> ()  [unwired: 1 in, 6 out]
        n146 = case shown="\"False\", Default" w173 {
          tunnel: [_ "wind speed updated"] -> w174
          frame "False", Default {
          }
          frame "wind-turbine" {
          }
        }
      }
      event "PA2": Value Change {
        n147 = event-data() -> ()  [unwired: 1 in, 6 out]
        n148 = case shown="\"False\", Default" w177 {
          tunnel: [_ "led flow speed updated"] -> w178
          frame "False", Default {
          }
          frame "wind-turbine" {
          }
        }
      }
      event "PA3": Value Change {
        n149 = event-data() -> ()  [unwired: 1 in, 6 out]
        n150 = case shown="\"wind-turbine\"" w181 {
          tunnel: [_ "pwm command updated"] -> w182
          frame "False", Default {
          }
          frame "wind-turbine" {
          }
        }
      }
      event "Reset Node": Value Change {
        n151 = event-data() -> ()  [unwired: 1 in, 6 out]
        n152 = case shown="\"wind-turbine\"" w185 {
          tunnel: [_ "reset to default"] -> w188
          tunnel: [_ "Enabled / Manual Ready"] -> w187
          tunnel: [_ "weather input"] -> w186
          frame "False", Default {
          }
          frame "wind-turbine" {
            n153 = local write "Node Enable"(TRUE ("Node Enable")) -> ()
            n154 = local write "PA2"(30.0 ("WT Wind Speed")) -> ()
            n155 = local write "PA1"(8.0 ("WT PWM Command")) -> ()
            n156 = local write "PA3"(80.0 ("WT PWM Command")) -> ()
          }
        }
      }
      event "Send UDP Command": Value Change {
        n157 = event-data() -> ()  [unwired: 1 in, 6 out]
        n158 = case shown="\"Load 1\"" w196 {
          tunnel: w202 -> [_ w209 _ _ _ _ _]
          tunnel: w201 -> [_ w204 _ _ _ _ _]
          tunnel: w200 -> [_ w205 _ _ _ _ _]
          tunnel: w199 -> [_ w208 _ _ _ _ _]
          tunnel: [_ w203 _ _ _ _ _] -> w198
          tunnel: [_ "command preview generated" _ _ _ _ _] -> w197
          frame "False", Default {
          }
          frame "wind-turbine" {
            n159 = call "BuildWindTurbineFrame.vi"("LED Flow Speed"=w208, "PWM Command"=w205, "Wind Speed"=w204, "Node Enable"=w209) -> ("Frame Preview"=w203:string)  [unwired: 1 out]
            n160 = call "SendUDP.vi"("Arg3"=w204, "IP"="192.168.10.81", "Port"=8008) -> ()  [unwired: 13 in]
          }
          frame "DESD 1" {
            w216 = 0
            n161 = local read "PA2"() -> (w214:dbl)
            n162 = local read "PA3"() -> (w213:dbl)
            n163 = local read "PA1"() -> (w211:dbl)
            n164 = Round To Nearest(number=w211) -> (nearest integer value=w212:dbl)
            n165 = call "SendUDP.vi"("Arg3"=w212, "IP"="192.168.10.51", "Port"=8008, "Arg4"=w214, "Arg5"=w213, "Arg6"=w216, "Arg7"=w216) -> ()  [unwired: 9 in]
          }
          frame "DESD 2 " {
            n166 = local read "PA2"() -> (w219:dbl)
            n167 = local read "PA1"() -> (w220:dbl)
            n168 = local read "PA3"() -> (w218:dbl)
            n169 = call "Sreen.vi"("IP"="192.168.10.52", "Voltage 2"=w218, "Voltage 1"=w219, "Battery"=w220) -> ()  [unwired: 1 in]
          }
          frame "DESD 3" {
            n170 = local read "PA2"() -> (w223:dbl)
            n171 = local read "PA1"() -> (w224:dbl)
            n172 = local read "PA3"() -> (w222:dbl)
            n173 = call "Sreen.vi"("IP"="192.168.10.53", "Voltage 2"=w222, "Voltage 1"=w223, "Battery"=w224) -> ()  [unwired: 1 in]
          }
          frame "DESD 4" {
            n174 = local read "PA2"() -> (w227:dbl)
            n175 = local read "PA1"() -> (w228:dbl)
            n176 = local read "PA3"() -> (w226:dbl)
            n177 = call "Sreen.vi"("IP"="192.168.10.54", "Voltage 2"=w226, "Voltage 1"=w227, "Battery"=w228) -> ()  [unwired: 1 in]
          }
          frame "Load 1" {
            w236 = 0
            w250 = "192.168.10.91"
            w249 = 8008
            n178 = local read "String Control"() -> (w245:string)
            n179 = local read "String Control"() -> (w248:string)
            n180 = String Subset(string=w245, offset (0)=8, length (rest)=8) -> (substring=w231:string)
            n181 = String Subset(string=w248, offset (0)=0, length (rest)=8) -> (substring=w242:string)
            n182 = String To Byte Array(string=w231) -> (unsigned byte array=w235:u8[])
            n183 = String To Byte Array(string=w242) -> (unsigned byte array=w241:u8[])
            n184 = Add(x=w235, y=-48) -> (x+y=w233:i32[])
            n185 = Add(x=w241, y=-48) -> (x+y=w239:i32[])
            n186 = Not Equal To 0?(x=w233) -> (x != 0?=w232:bool[])
            n187 = Not Equal To 0?(x=w239) -> (x != 0?=w238:bool[])
            n188 = Boolean Array To Number(Boolean array=w232) -> (number=w230:u32)
            n189 = Boolean Array To Number(Boolean array=w238) -> (number=w237:u32)
            n190 = call "SendUDP.vi"("Arg3"=w237, "IP"=w250, "Port"=w249, "Arg4"=w230, "Arg5"=w236, "Arg6"=w236, "Arg7"=w236) -> ()  [unwired: 9 in]
            "Port" <- w249
            "IP" <- w250
          }
        }
      }
      event "BTN_Wind_Turbine": Value Change {
        n191 = event-data() -> ()  [unwired: 1 in, 6 out]
        n192 = local write "Device Name"("WT 1 — Wind Turbine") -> ()
        n193 = local write "Device Badge"("weather input") -> ()
        n194 = local write "Local Status"("Enabled / Manual Ready") -> ()
        n195 = local write "Selected Summary"("Selected: WT 1") -> ()
        n196 = local write "Node ID"("windturbine-81") -> ()
        n197 = local write "Device Description"("P_min = 0 MW, P_max = 1.05 MW") -> ()
        n198 = property on="PA2" class="DigNum (strict)"("Caption.Text"="") -> ()  [unwired: 2 in, 2 out]
        n199 = property on="PA1" class="DigNum (strict)"("Caption.Text"="Wind Speed (m/s)") -> ()  [unwired: 2 in, 2 out]
        n200 = property on="PA3" class="DigNum (strict)"("Caption.Text"="") -> ()  [unwired: 2 in, 2 out]
      }
      event "Read Device State": Value Change {
        n201 = event-data() -> ()  [unwired: 1 in, 6 out]
        n202 = case shown="\"False\", Default" w262 {
          tunnel: [_ "telemetry updated locally"] -> w266
          tunnel: [_ "229.7"] -> w265
          tunnel: [_ "1.8"] -> w264
          tunnel: [_ "6.2"] -> w263
          frame "False", Default {
          }
          frame "wind-turbine" {
          }
        }
      }
      event "Mode 1：5-Day Rainstorm-to-Flood": Value Change {
        n203 = event-data() -> ()  [unwired: 1 in, 6 out]
        n204 = Read from Text File(file (use dialog)=path "/Users/johnnychao/Documents/ENGR4903J/project/led_test.txt") -> (text=w271:string)  [unwired: 3 in, 3 out]
        n205 = while {
          shift-right: [w275] -> _
          shift-left: w271 -> [w286]
          i -> [w273]
          stop <- w274 stop-if-true
          n206 = Match Pattern(string=w286, regular expression="\\n") -> (before substring=w276:string, after substring=w275:string)  [unwired: 1 in, 2 out]
          "after substring" <- w275
          n207 = call <vilib>:"Trim Whitespace.vi"("string"=w276) -> ("trimmed string"=w281:string)  [unwired: 1 in]
          n208 = Match Pattern(string=w276, regular expression="#") -> (before substring=w283:string)  [unwired: 1 in, 3 out]
          n209 = String Length(string=w281) -> (length=w280:i32)
          n210 = Equal To 0?(x=w280) -> (x = 0?=w278:bool)
          n211 = Equal?(x=w283, y="" ("regular expression")) -> (x = y?=w279:bool)
          n212 = Or(x=w279, y=w278) -> (x .or. y?=w277:bool)
          n213 = case shown="False" w277 {
            tunnel: w276 -> [w293 _]
            frame False {
              n214 = Scan From String "Scan From String"(format string="LED %d", input string=w293) -> (remaining string=w300:string, output 1=w301:i32)  [unwired: 3 in, 2 out]
              n215 = Scan From String(format string=" color=%d", input string=w300) -> (remaining string=w291:string, output 1=w303:u8)  [unwired: 3 in, 2 out]
              n216 = Scan From String(format string=", bright=%d", input string=w291) -> (remaining string=w290:string, output 1=w304:u8)  [unwired: 3 in, 2 out]
              n217 = Scan From String(format string=", speed=%d", input string=w290) -> (output 1=w289:u8)  [unwired: 3 in, 3 out]
              n218 = local write "script Status 2"(w290) -> ()
              n219 = Add(x=w301, y=0) -> (x+y=w302:i32)
              n220 = Format Into String(format string="192.168.10.%d", w302) -> (resulting string=w305:string)  [unwired: 2 in, 1 out]
              n221 = call "LED.vi"("Speed"=w289, "IP"=w305, "Length"=1, "Brightness"=w304, "Color"=w303, "Direction"=1) -> ()  [unwired: 2 in]
            }
            frame True {
            }
          }
          n222 = local write "remaining text"(w275) -> ()
          n223 = String Length(string=w275) -> (length=w285:i32)
          n224 = Equal To 0?(x=w285) -> (x = 0?=w274:bool)
          n225 = local write "script Status"(w276) -> ()
          "String" <- w286
          "Numeric" <- w273
        }
      }
      event "Mode 2": Value Change {
        n226 = event-data() -> ()  [unwired: 1 in, 6 out]
        n227 = Read from Text File(file (use dialog)=path "D:/learn/led_test.txt") -> (text=w306:string)  [unwired: 3 in, 3 out]
        n228 = Match Pattern(string=w306, regular expression="\\n") -> (before substring=w308:string, after substring=w307:string)  [unwired: 1 in, 2 out]
        n229 = call <vilib>:"Trim Whitespace.vi"("string"=w308) -> ("trimmed string"=w313:string)  [unwired: 1 in]
        n230 = Match Pattern(string=w308, regular expression="#") -> (before substring=w315:string)  [unwired: 1 in, 3 out]
        n231 = String Length(string=w313) -> (length=w312:i32)
        n232 = Equal To 0?(x=w312) -> (x = 0?=w310:bool)
        n233 = Equal?(x=w315, y="" ("regular expression")) -> (x = y?=w311:bool)
        n234 = Or(x=w311, y=w310) -> (x .or. y?=w309:bool)
        n235 = case shown="False" w309 {
          tunnel: w308 -> [w322 _]
          frame False {
            n236 = Scan From String "Scan From String"(format string="LED %d", input string=w322) -> (remaining string=w329:string, output 1=w331:i32)  [unwired: 3 in, 2 out]
            n237 = Scan From String(format string=" color=%d", input string=w329) -> (remaining string=w320:string, output 1=w333:u8)  [unwired: 3 in, 2 out]
            n238 = Scan From String(format string=", bright=%d", input string=w320) -> (remaining string=w330:string, output 1=w334:u8)  [unwired: 3 in, 2 out]
            n239 = Scan From String(format string=", speed=%d", input string=w330) -> (output 1=w335:u8)  [unwired: 3 in, 3 out]
            n240 = Add(x=w331, y=0) -> (x+y=w332:i32)
            n241 = Format Into String(format string="192.168.10.%d", w332) -> (resulting string=w336:string)  [unwired: 2 in, 1 out]
            n242 = call "LED.vi"("IP"=w336, "Length"=w335, "Brightness"=w334, "Color"=w333, "Direction"=1) -> ()  [unwired: 3 in]
          }
          frame True {
          }
        }
        n243 = String Length(string=w307) -> (length=w317:i32)
        n244 = Equal To 0?(x=w317) -> ()  [unwired: 1 out]
      }
      event "stop": Value Change {
        n245 = event-data() -> ()  [unwired: 1 in, 6 out]
      }
    }
    "Last Update" <- w16
    "UDP Frame" <- w11
    "Voltage" <- w10
    "Current" <- w9
    "Active Power" <- w8
  }
